vi "failUnlessXmlGeneratedCorrectly.vi"(4 "Convert EOL? (TRUE)":bool=TRUE, 6 "message (\"\")":string, 8 "error in":errorcluster, 9 "expected XML string":string, 10 "Input Data":variant, 11 "EasyXMLTest in":refnum<class "EasyXMLTest.lvclass">) -> (0 "error out":errorcluster, 2 "Generated XML String":string, 3 "EasyXMLTest out":refnum<class "EasyXMLTest.lvclass">)   [LabVIEW 2011, in "EasyXMLTest.lvclass"]
uses:
  EasyXMLTest.lvclass
panel:
  # "Copyright © 2007 James Kring, Inc. All rights reserved.\n\nAuthor: Jim Kring [jim.kring@jameskring.com]\n\nThis library is provided \"AS IS\" ,WITHOUT WARRANTIES OR \nCONDITIONS OF ANY KIND, either express or implied.\n\nJames Kring, Inc. -- http://www.jameskring.com"
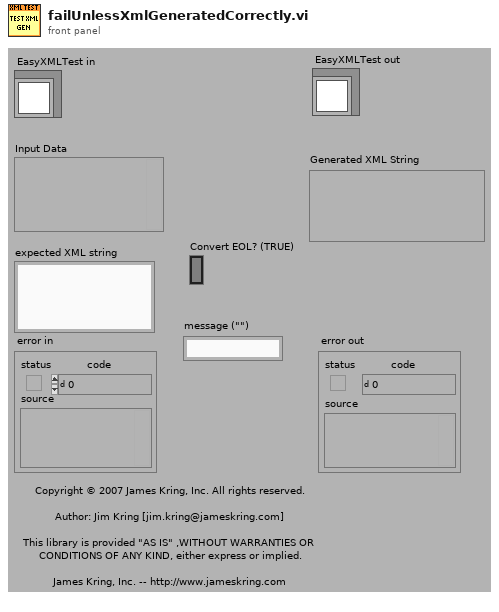
[diagram p1: front panel]
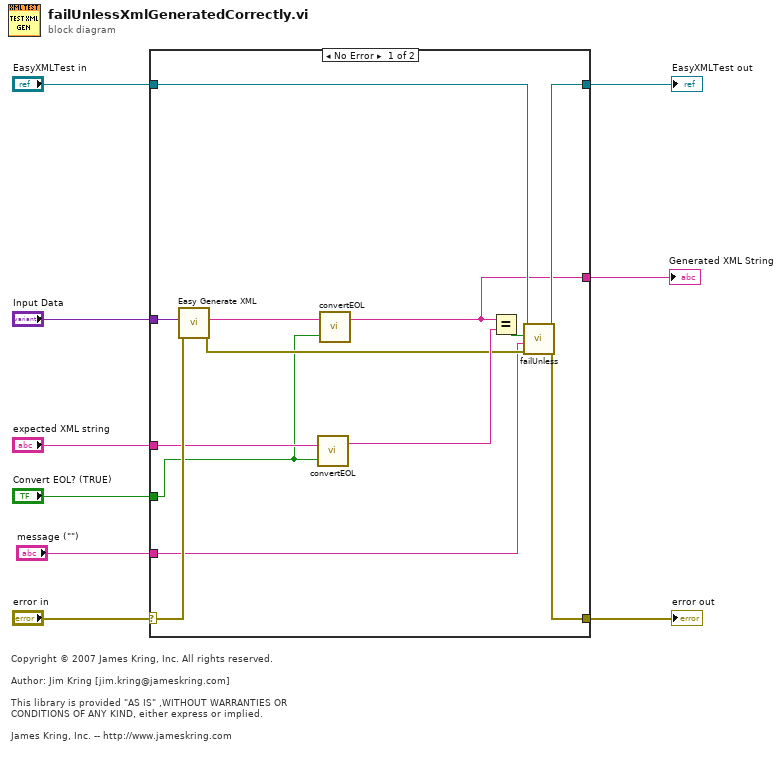
[diagram p0: block diagram]
diagram:
  # "Copyright © 2007 James Kring, Inc. All rights reserved.\n\nAuthor: Jim Kring [jim.kring@jameskring.com]\n\nThis library is provided \"AS IS\" ,WITHOUT WARRANTIES OR \nCONDITIONS OF ANY KIND, either express or implied.\n\nJames Kring, Inc. -- http://www.jameskring.com"
  n1 = case shown="No Error" "error in" {
    selector: "error in" -> [w21 w24]
    tunnel: [w16 w24] -> w4
    tunnel: "EasyXMLTest in" -> [w18 w23]
    tunnel: [w17 w23] -> w6
    tunnel: "Input Data" -> [w22 _]
    tunnel: "expected XML string" -> [w20 _]
    tunnel: "message (\"\")" -> [w13 _]
    tunnel: [w10 _] -> w2
    tunnel: "Convert EOL? (TRUE)" -> [w12 _]
    frame No Error {
      n2 = call "Easy Generate XML.vi"("error in (no error)"=w21, "LabVIEW Data"=w22) -> ("error out"=w15:errorcluster, "XML String"=w11:string)  [unwired: 8 in]
      n3 = call "convertEOL.vi"("Convert EOL? (TRUE)"=w12, "string"=w20) -> ("string out"=w19:string)  [unwired: 1 in]
      n4 = call "convertEOL.vi"("Convert EOL? (TRUE)"=w12, "string"=w11) -> ("string out"=w10:string)  [unwired: 1 in]
      n5 = Equal?(x=w10, y=w19) -> (x = y?=w14:bool)
      n6 = call-dynamic "failUnless.vi"("error in (no error)"=w15, "message (\"\")"=w13, "pass"=w14, "TestCase in"=w18) -> ("error out"=w16:errorcluster, "TestCase out"=w17:refnum<class "EasyXMLTest.lvclass">)  [unwired: 6 in]
    }
    frame Error {
    }
  }
  "EasyXMLTest out" <- w6
  "error out" <- w4
  "Generated XML String" <- w2
